vi "Generate Thetas.vi"(8 "y unflat":cluster{dbl[]}[](array[cluster]), 9 "ctrl pts":cluster{sgl, sgl}[][](array[cluster]), 10 "starting angle":sgl, 11 "spline flat":cluster{"x":sgl, "y":sgl}[](array[cluster])) -> (1 "Tangent Vector":cluster{"x out":dbl, "y out":dbl}[](array[cluster]), 2 "theta":sgl[](array[numeric]), 3 "omega":sgl[](array[numeric]))   [LabVIEW 2023]
panel:
  in  "dt":sgl
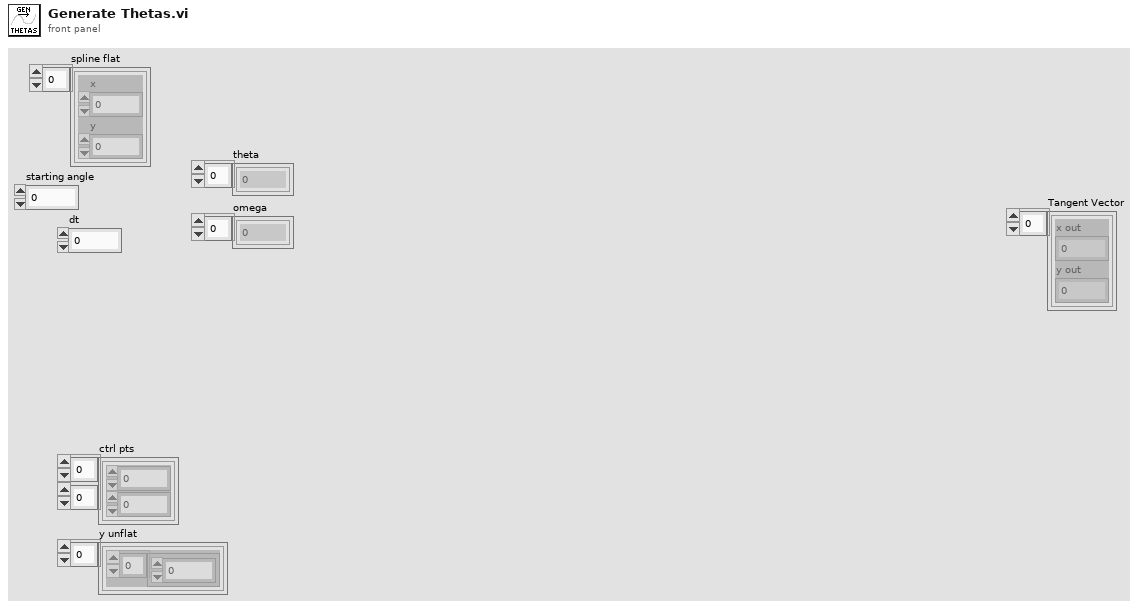
[diagram p1: front panel]
types:
  T1 = typedef "Bezier Curve.ctl" = cluster{"x":sgl, "y":sgl}[]
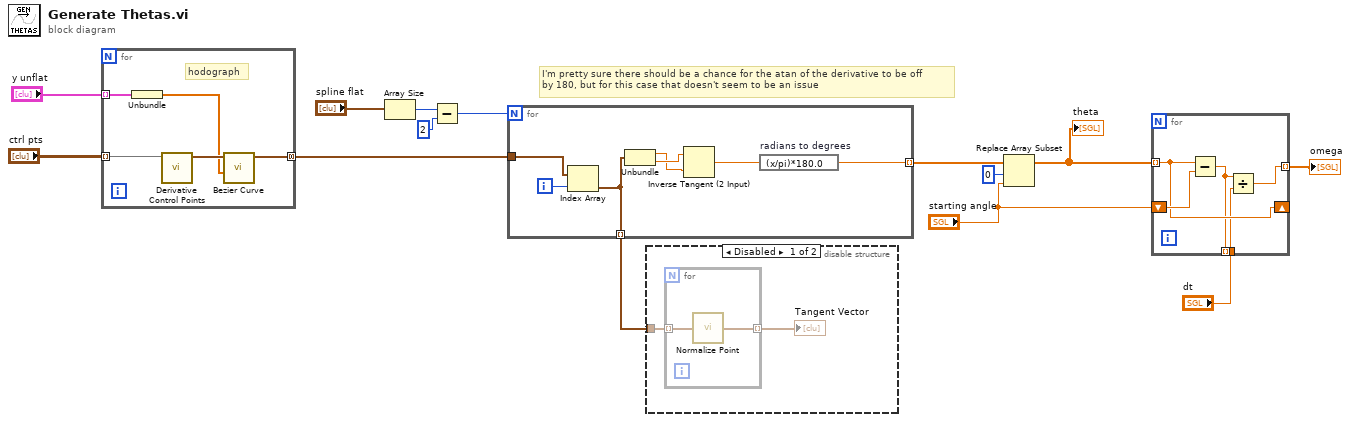
[diagram p0: block diagram]
diagram:
  # "I'm pretty sure there should be a chance for the atan of the derivative to be off\nby 180, but for this case that doesn't seem to be an issue"
  n1 = for {
    tunnel: "ctrl pts" -> [w19] mode=indexing
    tunnel: "y unflat" -> [w17] mode=indexing
    tunnel: [w15] -> w5 mode=concatenating
    # "hodograph"
    n2 = Unbundle(w17) -> (w16:dbl[])
    n3 = call "Derivative Control Points.vi"("ctrl points"=w19) -> ("d ctrl pts"=w18:cluster{dbl, dbl}[])  [unwired: 10 in]
    n4 = call "Bezier Curve.vi"("position"=w16, "ctrl points"=w18) -> ("curve"=w15:T1)  [unwired: 8 in, 1 out]
  }
  n5 = Array Size(array="spline flat") -> (size(s)=w14:i32)
  n6 = Subtract(x=w14, y=2) -> (x-y=w12:i32)
  n7 = for {
    N: w12 -> [_]
    tunnel: w5 -> [w22]
    tunnel: [w23] -> w11 mode=indexing
    tunnel: [w20] -> w1 mode=indexing
    i -> [w21]
    n8 = Index Array(array=w22, index=w21) -> (element=w20:cluster{"x":sgl, "y":sgl})
    n9 = Unbundle(w20) -> ("x"=w25:sgl, "y"=w26:sgl)
    n10 = Inverse Tangent (2 Input)(1:w25, 2:w26) -> (0:w24:sgl)
    n11 = expression code="(x/pi)*180.0" "radians to degrees"(w24) -> (w23:sgl)
  }
  n12 = disable-structure shown="Disabled" {
    disable-tunnel: w1 -> [w28 _]
    frame Disabled {
      n13 = for {
        tunnel: w28 -> [w29] mode=indexing
        tunnel: [w30] -> w27 mode=indexing
        n14 = call "Normalize Point.vi"("point in"=w29) -> ("point out"=w30:cluster{"x":sgl, "y":sgl})
      }
      "Tangent Vector" <- w27
    }
    frame Enabled {
    }
  }
  n15 = Replace Array Subset(array=w11, new element="starting angle", index=0) -> (w2:sgl[])
  "theta" <- w2
  n16 = for {
    tunnel: w2 -> [w34] mode=indexing
    shift-right: [w34] -> _
    shift-left: "starting angle" -> [w35]
    tunnel: [w32] -> w8 mode=indexing
    tunnel: "dt" -> [w33]
    tunnel: [w31] -> _ mode=indexing
    n17 = Subtract(x=w34, y=w35) -> (x-y=w31:sgl)
    n18 = Divide(x=w31, y=w33) -> (x/y=w32:sgl)
  }
  "omega" <- w8
